vi "kernel32 QueryFullProcessImageNameW.vi"(0 "hProcess":u64, 5 "size":u32=1024, 7 "dwFlags":u32, 11 "error in":errorcluster) -> (4 "path":u16[](array[numeric]), 6 "return value":i32, 15 "error out":errorcluster)   [LabVIEW 2020, in "RemoteVI.lvlib"]
doc: "Returns the full path of the program a process runs, as UTF-16 code units, through kernel32.dll QueryFullProcessImageNameW (stdcall, called in any thread). hProcess comes from kernel32 OpenProcess.vi with PROCESS_QUERY_LIMITED_INFORMATION. The buffer is size code units of zeros and the path is cut at its terminating 0. return value is the Win32 BOOL: non-zero on success. When error in carries an error the DLL is not called. Generated by scripts\\Build Win32 Wrappers.vi - do not edit by hand, rebuild it."
uses:
  RemoteVI.lvlib
  kernel32.dll
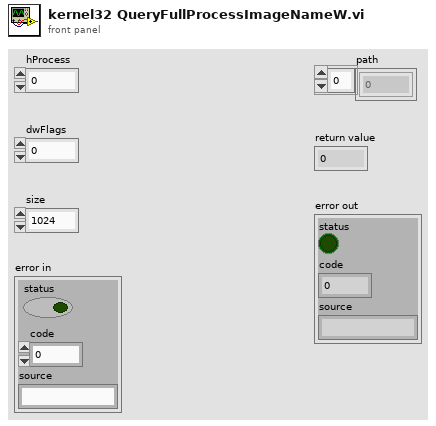
[diagram p1: front panel]
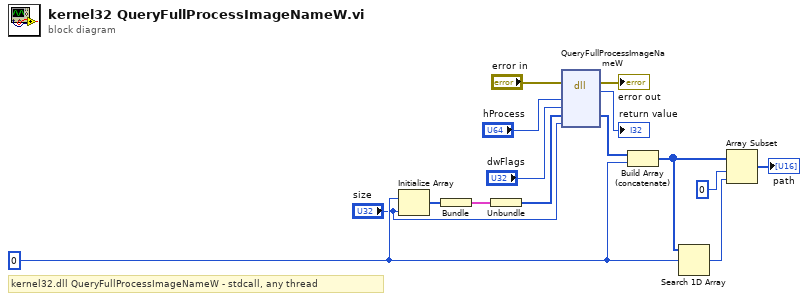
[diagram p0: block diagram]
diagram:
  w10 = u16 0
  # "kernel32.dll QueryFullProcessImageNameW - stdcall, any thread"
  n1 = Initialize Array(w10, "size") -> (w11:u16[])
  n2 = Bundle(w11) -> (w12:cluster{u16[]})  [unwired: 1 in]
  n3 = Unbundle(w12) -> (w2:u16[])
  n4 = dll-call lib="kernel32.dll" fn="QueryFullProcessImageNameW"(error in="error in", "hProcess"="hProcess", "dwFlags"="dwFlags", "lpExeName"=w2, "lpdwSize"="size") -> (error out=→"error out":errorcluster, →"return value":i32, "lpExeName"=w1:u16[])  [unwired: 5 in, 1 out]
  n5 = Build Array (concatenate)(w1, w10) -> (w13:u16[])
  n6 = Search 1D Array(1D array=w13, element=w10) -> (index of element=w14:i32)  [unwired: 1 in]
  n7 = Array Subset(array=w13, index=0, length=w14) -> (→"path":u16[])
